vi "Timeout.vi"(8 "error in (no error)":errorcluster, 11 "object in":refnum<class "ChannelManagerUI.lvclass">) -> (0 "error out":errorcluster, 3 "object out":refnum<class "ChannelManagerUI.lvclass">)   [LabVIEW 2021, in "Channel.lvlib" / "ChannelManagerUI.lvlib" / "ChannelManagerUI.lvclass"]
uses:
  ChannelManagerUI.lvclass
  Channel_class/Channel.lvclass
  ChannelManagerUI.lvclass/ChannelManagerUI.ctl
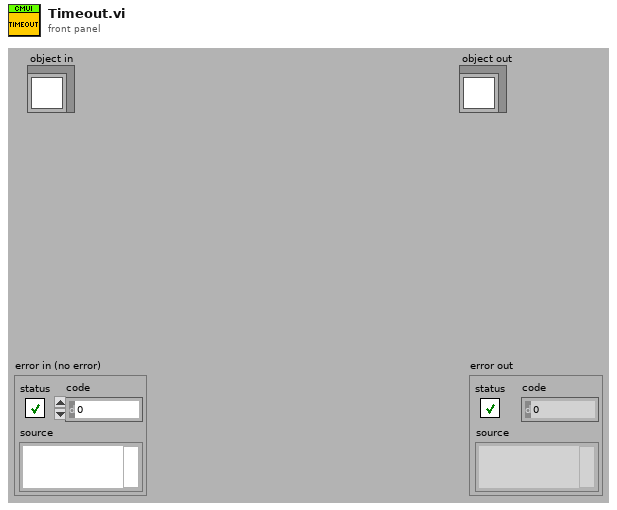
[diagram p1: front panel]
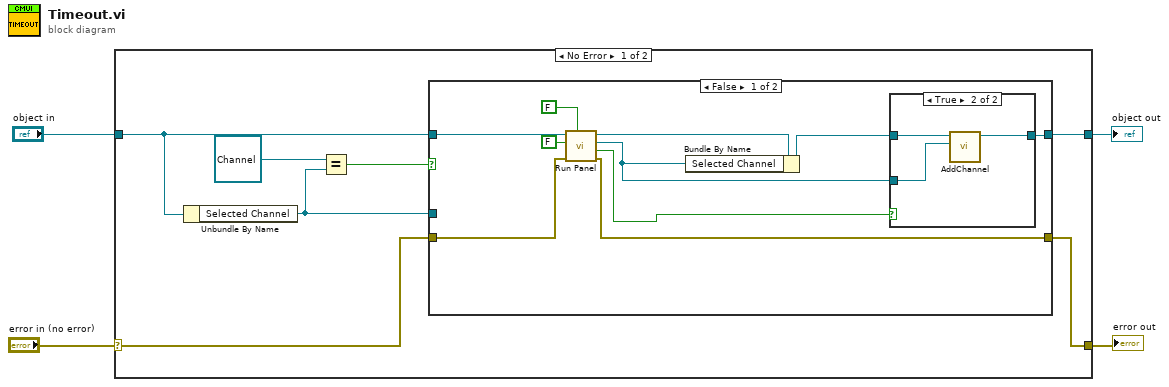
[diagram p0: block diagram]
diagram:
  n1 = case shown="No Error" "error in (no error)" {
    selector: "error in (no error)" -> [w6 w29]
    tunnel: [w7 w29] -> w3
    tunnel: [w9 w28] -> w1
    tunnel: "object in" -> [w8 w28]
    frame No Error {
      n2 = Unbundle By Name(w8) -> ("Selected Channel"=w10:refnum<class "Channel.lvclass">)
      n3 = Equal?(x=refnum<class "Channel.lvclass"> refnum ("y"), y=w10) -> (x = y?=w5:bool)
      n4 = case shown="False" w5 {
        tunnel: w10 -> [_ _]
        tunnel: [w20 w27] -> w9
        tunnel: w8 -> [w21 w27]
        tunnel: [w15 w26] -> w7
        tunnel: w6 -> [w14 w26]
        frame False {
          n5 = call "Run Panel.vi"("Set(F)"=FALSE, "error in (no error)"=w14, "First Time(F)"=FALSE, "ChannelManagerUI in"=w21) -> ("error out"=w15:errorcluster, "Changed?"=w16:bool, "Channel"=w17:refnum<class "Channel.lvclass">, "ChannelManagerUI out"=w18:refnum<class "ChannelManagerUI.lvclass">)  [unwired: 4 in]
          n6 = Bundle By Name(cluster=w18, "Selected Channel"=w17) -> (w19:refnum<class "ChannelManagerUI.lvclass">)
          n7 = case shown="True" w16 {
            tunnel: [w22 w24] -> w20
            tunnel: w19 -> [w22 w25]
            tunnel: w17 -> [_ w23]
            frame False {
            }
            frame True {
              n8 = call-dynamic "AddChannel.vi"("Channel"=w23, "object in"=w25) -> ("object out"=w24:refnum<class "ChannelManagerUI.lvclass">)  [unwired: 8 in, 1 out]
            }
          }
        }
        frame True {
        }
      }
    }
    frame Error {
    }
  }
  "error out" <- w3
  "object out" <- w1
